vi "VIH Utility - STR - Match Pattern - Find at Minimum Position.vi"(8 "offset (0)":i32, 9 "case-sensitive (F)":bool, 10 "Regular expressions":string[](array[string]), 11 "String":string) -> (0 "offset past match":i32, 1 "after substring":string, 2 "match substring":string, 3 "before substring":string, 5 "first match index":i32)   [LabVIEW 2014]
doc: "::: VI Helpeks :::\nCopyright (c) 2000-2026 Konstantin Shifershteyn. All rights reserved."
panel:
  # "VI Helpeks\nCopyright (c) 2012-2026 Konstantin Shifershteyn"
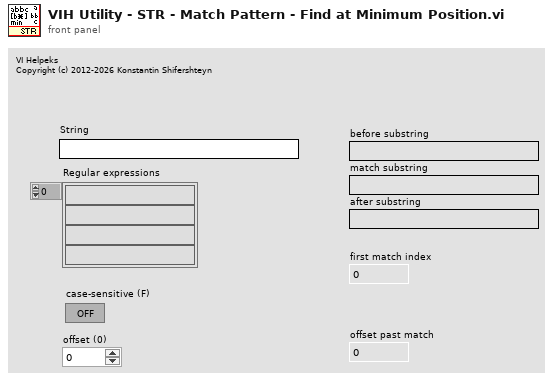
[diagram p1: front panel]
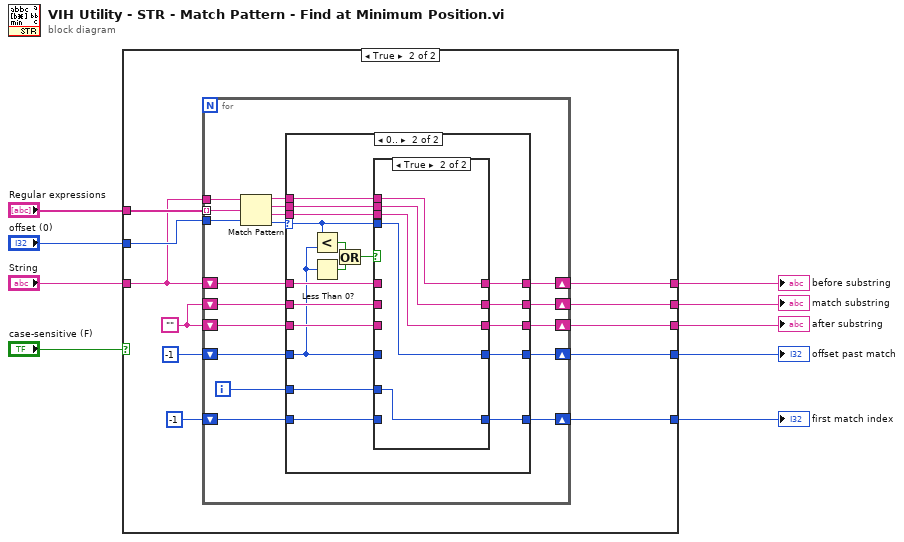
[diagram p0: block diagram]
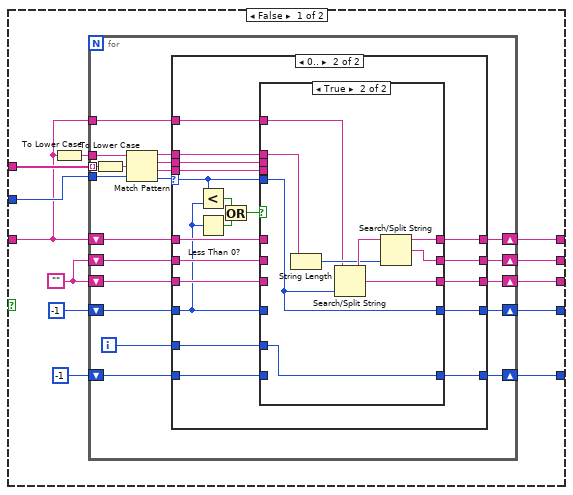
[diagram p2: hidden frame]
diagram:
  n1 = case shown="True" "case-sensitive (F)" {
    tunnel: "Regular expressions" -> [w21 w90]
    tunnel: [w20 w89] -> w8
    tunnel: [w17 w86] -> w7
    tunnel: [w16 w85] -> w6
    tunnel: [w15 w84] -> w5
    tunnel: [w14 w83] -> w4
    tunnel: "offset (0)" -> [w13 w82]
    tunnel: "String" -> [w11 w80]
    frame False {
      w19 = ""
      n2 = To Lower Case(string=w11) -> (all lower case string=w10:string)
      n3 = for {
        shift-right: [w26] -> w20
        shift-left: -1 -> [w24]
        tunnel: w10 -> [w41]
        tunnel: w21 -> [w40] mode=indexing
        shift-right: [w37] -> w16
        shift-left: w11 -> [w36]
        shift-right: [w35] -> w15
        shift-left: w19 -> [w34]
        shift-right: [w33] -> w14
        shift-left: w19 -> [w32]
        shift-right: [w31] -> w17
        shift-left: -1 ("offset past match") -> [w30]
        tunnel: w13 -> [w39]
        tunnel: w11 -> [w23]
        i -> [w25]
        n4 = To Lower Case(string=w40) -> (all lower case string=w22:string)
        n5 = Match Pattern(string=w41, regular expression=w22, offset (0)=w39) -> (before substring=w29:string, match substring=w28:string, after substring=w27:string, offset past match=w38:i32)
        n6 = case shown="0.." w38 {
          selector: w38 -> [_ w55]
          tunnel: [w46 w62] -> w37
          tunnel: w36 -> [w46 w52]
          tunnel: [w45 w60] -> w35
          tunnel: w34 -> [w45 w51]
          tunnel: [w44 w58] -> w33
          tunnel: w32 -> [w44 w50]
          tunnel: [w43 w56] -> w31
          tunnel: w30 -> [w43 w49]
          tunnel: w29 -> [_ w61]
          tunnel: w28 -> [_ w59]
          tunnel: w27 -> [_ w57]
          tunnel: [w42 w54] -> w26
          tunnel: w25 -> [_ w53]
          tunnel: w24 -> [w42 w48]
          tunnel: w23 -> [_ w47]
          frame ..-1 {
          }
          frame 0.. {
            n7 = Less?(x=w55, y=w49) -> (x < y?=w64:bool)
            n8 = Less Than 0?(x=w49) -> (x < 0?=w65:bool)
            n9 = Or(x=w64, y=w65) -> (x .or. y?=w63:bool)
            n10 = case shown="True" w63 {
              tunnel: [w70 w72] -> w62
              tunnel: w61 -> [_ w77]
              tunnel: [w69 w73] -> w60
              tunnel: w59 -> [_ _]
              tunnel: [w68 w74] -> w58
              tunnel: w57 -> [_ _]
              tunnel: [w67 w78] -> w56
              tunnel: w55 -> [_ w78]
              tunnel: [w66 w79] -> w54
              tunnel: w53 -> [_ w79]
              tunnel: w52 -> [w70 _]
              tunnel: w51 -> [w69 _]
              tunnel: w50 -> [w68 _]
              tunnel: w49 -> [w67 _]
              tunnel: w48 -> [w66 _]
              tunnel: w47 -> [_ w71]
              frame False {
              }
              frame True {
                n11 = String Length(string=w77) -> (length=w75:i32)
                n12 = Search/Split String(string=w71, offset (0)=w78) -> (substring before match=w76:string, match + rest of string=w74:string)  [unwired: 1 in, 1 out]
                n13 = Search/Split String(string=w76, offset (0)=w75) -> (substring before match=w72:string, match + rest of string=w73:string)  [unwired: 1 in, 1 out]
              }
            }
          }
        }
      }
    }
    frame True {
      w88 = ""
      n14 = for {
        shift-right: [w94] -> w89
        shift-left: -1 -> [w92]
        tunnel: w80 -> [w108]
        tunnel: w90 -> [w91] mode=indexing
        shift-right: [w105] -> w85
        shift-left: w80 -> [w104]
        shift-right: [w103] -> w84
        shift-left: w88 -> [w102]
        shift-right: [w101] -> w83
        shift-left: w88 -> [w100]
        shift-right: [w99] -> w86
        shift-left: -1 ("offset past match") -> [w98]
        tunnel: w82 -> [w107]
        i -> [w93]
        n15 = Match Pattern(string=w108, regular expression=w91, offset (0)=w107) -> (before substring=w97:string, match substring=w96:string, after substring=w95:string, offset past match=w106:i32)
        n16 = case shown="0.." w106 {
          selector: w106 -> [_ w121]
          tunnel: [w113 w128] -> w105
          tunnel: w104 -> [w113 w118]
          tunnel: [w112 w126] -> w103
          tunnel: w102 -> [w112 w117]
          tunnel: [w111 w124] -> w101
          tunnel: w100 -> [w111 w116]
          tunnel: [w110 w122] -> w99
          tunnel: w98 -> [w110 w115]
          tunnel: w97 -> [_ w127]
          tunnel: w96 -> [_ w125]
          tunnel: w95 -> [_ w123]
          tunnel: [w109 w120] -> w94
          tunnel: w93 -> [_ w119]
          tunnel: w92 -> [w109 w114]
          frame ..-1 {
          }
          frame 0.. {
            n17 = Less?(x=w121, y=w115) -> (x < y?=w130:bool)
            n18 = Less Than 0?(x=w115) -> (x < 0?=w131:bool)
            n19 = Or(x=w130, y=w131) -> (x .or. y?=w129:bool)
            n20 = case shown="True" w129 {
              tunnel: [w136 w137] -> w128
              tunnel: w127 -> [_ w137]
              tunnel: [w135 w138] -> w126
              tunnel: w125 -> [_ w138]
              tunnel: [w134 w139] -> w124
              tunnel: w123 -> [_ w139]
              tunnel: [w133 w140] -> w122
              tunnel: w121 -> [_ w140]
              tunnel: [w132 w141] -> w120
              tunnel: w119 -> [_ w141]
              tunnel: w118 -> [w136 _]
              tunnel: w117 -> [w135 _]
              tunnel: w116 -> [w134 _]
              tunnel: w115 -> [w133 _]
              tunnel: w114 -> [w132 _]
              frame False {
              }
              frame True {
              }
            }
          }
        }
      }
    }
  }
  "first match index" <- w8
  "offset past match" <- w7
  "before substring" <- w6
  "match substring" <- w5
  "after substring" <- w4
